vi "FuncVI-Abort.vi"(5 "InstanceRef":T2, 9 "arg list":T1[](array[typedef]) {"num" format="%.2f"}) -> (0 "error out":bool, 3 "result":T1 {"num" format="%.2f"})   [LabVIEW 2021]
doc: "::: CalcExpress Toolkit :::\nCopyright (c) 2000-2026 Konstantin Shifershteyn. All rights reserved."
uses:
  cetypes.llb/CalcExpress Function Argument Info.ctl
  cetypes.llb/CalcExpress Instance RefNum.ctl
panel:
  in  "max arg num":i32
  in  "min arg num":i32
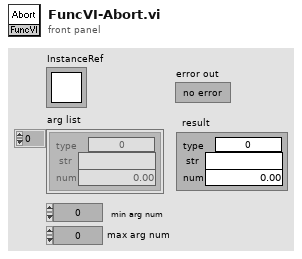
[diagram p1: front panel]
types:
  T1 = typedef "CalcExpress Function Argument Info.ctl" = cluster{"type":u32, "str":string, "num":dbl}
  T2 = typedef "CalcExpress Instance RefNum.ctl" = refnum<k1>
  T3 = cluster{"use this constant to specify a predefined type":enum32{"String", "DBL Number", "identifier", "1D Array of DBL", "2D Array of DBL", "CDB Number", "1D Array of CDB", "2D Array of CDB", "1D Array of String", "2D Array of String", "Unknown data type"}, string, "numeric value":dbl}
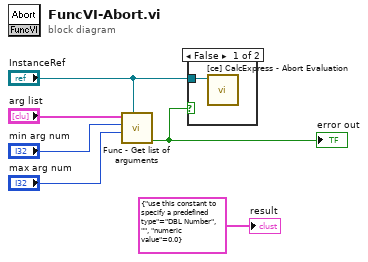
[diagram p0: block diagram]
diagram:
  n1 = call "Func - Get list of arguments.vi"("InstanceRef"="InstanceRef", "max arg num"="max arg num", "min arg num"="min arg num", "arg list"="arg list") -> ("error out"=w1:bool)  [unwired: 4 in, 3 out]
  "error out" <- w1
  n2 = case shown="False" w1 {
    tunnel: "InstanceRef" -> [w7 _]
    frame False {
      n3 = call "[ce] CalcExpress - Abort Evaluation.vi"("CE InstanceRef"=w7) -> ()  [unwired: 7 in, 2 out]
    }
    frame True {
    }
  }
  "result" <- T3 {"use this constant to specify a predefined type"=enum."DBL Number", "", "numeric value"=0.0}
